vi "GetImage.vi"(0 "XRef":T6, 1 "State In":T3) -> (14 "Image":T2, 15 "Fatal Error Out":T1)   [LabVIEW 2021, in "FirstXNode .xnode"]
uses:
  FirstXNode .xnode
  <vilib>/XNodeSupport/XNodeXNodeRef.ctl
  State.ctl
  <vilib>/XNodeSupport/XNodeBounds.ctl
  <vilib>/XNodeSupport/XNodeInt.ctl
  <vilib>/XNodeSupport/XNodeImage.ctl
  <vilib>/XNodeSupport/XNodeErrorCluster.ctl
  <vilib>/Utility/Data Type/Type Definitions/Data Type.ctl
  <vilib>/XNodeSupport/NI_XNodeSupport.lvlib
  <vilib>/Utility/Data Type/NI_Data Type.lvlib
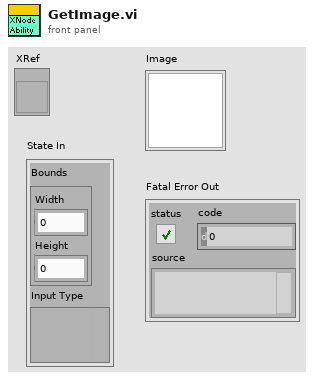
[diagram p1: front panel]
types:
  T1 = typedef "NI_XNodeSupport.lvlib/XNodeErrorCluster.ctl" = errorcluster
  T2 = typedef "NI_XNodeSupport.lvlib/XNodeImage.ctl" = picture
  T3 = typedef "FirstXNode .xnode/State.ctl" = cluster{"Bounds":T4, "Input Type":variant}
  T4 = typedef "NI_XNodeSupport.lvlib/XNodeBounds.ctl" = cluster{"Width":T5, "Height":T5}
  T5 = typedef "NI_XNodeSupport.lvlib/XNodeInt.ctl" = i32
  T6 = typedef "NI_XNodeSupport.lvlib/XNodeXNodeRef.ctl" = refnum<vi>
  T7 = typedef "NI_Data Type.lvlib/Data Type.ctl" = enum8{"Invalid Type", "Void", "I8", "I16", "I32", "I64", "U8", "U16", "U32", "U64", "Single Float", "Double Float", "Extended Float", "Single Complex", "Double Complex", "Extended Complex", "Enum U8", "Enum U16", "Enum U32", "Enum U64", "Single Float With Unit", "Double Float With Unit", "Extended Float With Unit", "Single Complex with Unit", "Double Complex with Unit", "Extended Complex with Unit", "Boolean", "String", "Path", "Picture", "Tag", "Array", "Cluster", "Variant", "LV Variant", "Waveform", "Timestamp", "Digital Waveform", "Digital Data", "ExpressData", "Refnum", "External Data", "VI", "Poly VI", "LabVIEW Class Instance", "Fixed Point", "Set Collection", "Map Collection"}
  T8 = enum32{"Solid", "Dash", "Dot", "DashDot", "DashDotDot"}
  T9 = cluster{"Width":T5, "Style":enum32{"Solid", "Dash", "Dot", "DashDot", "DashDotDot"}}
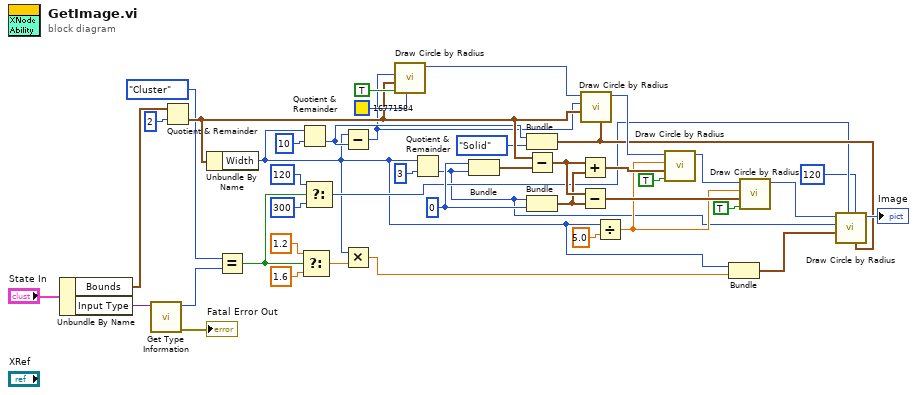
[diagram p0: block diagram]
diagram:
  w26 = i16 0 ("horizontal")
  n1 = Unbundle By Name("State In") -> ("Bounds"=w30:T4, "Input Type"=w14:variant)
  n2 = call <vilib>:"Get Type Information.vi"("variant"=w14) -> ("error out"=→"Fatal Error Out":errorcluster, "type"=w1:T7)  [unwired: 6 in, 3 out]
  n3 = Quotient & Remainder(x=w30, y=T5 2) -> (floor(x/y)=w29:T4)  [unwired: 1 out]
  n4 = Unbundle By Name(w29) -> ("Width"=w4:T5)
  n5 = Equal?(x=Data_Type."Cluster", y=w1) -> (x = y?=w8:bool)
  n6 = Quotient & Remainder(x=w4, y=T5 10) -> (floor(x/y)=w16:T5)  [unwired: 1 out]
  n7 = Select(t=1.2, s=w8, f=1.6 ("y")) -> (s? t:f=w11:dbl)
  n8 = Select(t=i16 120 ("start angle(0)"), s=w8, f=i16 300 ("start angle(0)")) -> (s? t:f=w9:i16)
  n9 = Subtract(x=w4, y=w16) -> (x-y=w15:T5)
  n10 = Multiply(x=w4, y=w11) -> (x*y=w23:dbl)
  n11 = call <vilib>:"Draw Circle by Radius.vi"("color(black)"=u32 16771584, "fill?(F)"=TRUE, "pixel center"=w29, "radius"=w15) -> ("new picture"=w41:picture)  [unwired: 7 in]
  n12 = Quotient & Remainder(x=w4, y=T5 3) -> (floor(x/y)=w3:T5)  [unwired: 1 out]
  n13 = Bundle("horizontal"=w26, "Width"=w3) -> (w27:cluster{"horizontal":i16, "Width":T5})  [unwired: 1 in]
  n14 = Bundle("Width"=w16, "Style"=T8."Solid") -> (w17:T9)  [unwired: 1 in]
  n15 = Subtract(x=w29, y=w27) -> (x-y=w36:T4)
  n16 = Bundle("Width"=w3, "horizontal"=w26) -> (w25:cluster{"Width":T5, "horizontal":i16})  [unwired: 1 in]
  n17 = Add(x=w36, y=w25) -> (x+y=w38:T4)
  n18 = Subtract(x=w36, y=w25) -> (x-y=w35:T4)
  n19 = call <vilib>:"Draw Circle by Radius.vi"("pen"=w17, "pixel center"=w29, "radius"=w15, "picture"=w41) -> ("new picture"=w40:picture)  [unwired: 7 in]
  n20 = Divide(x=w4, y=5.0) -> (x/y=w20:dbl)
  n21 = call <vilib>:"Draw Circle by Radius.vi"("fill?(F)"=TRUE, "pixel center"=w38, "radius"=w20, "picture"=w40) -> ("new picture"=w37:picture)  [unwired: 7 in]
  n22 = Bundle("Width"=w4, w23) -> (w24:cluster{"Width":T5, dbl})  [unwired: 1 in]
  n23 = call <vilib>:"Draw Circle by Radius.vi"("fill?(F)"=TRUE, "pixel center"=w35, "radius"=w20, "picture"=w37) -> ("new picture"=w33:picture)  [unwired: 7 in]
  n24 = call <vilib>:"Draw Circle by Radius.vi"("pen"=w17, "arc size(360)"=i16 120, "start angle(0)"=w9, "pixel center"=w24, "radius"=w3, "picture"=w33) -> ("new picture"=→"Image":picture)  [unwired: 5 in]
